vi "FuncVI_Sub - Script - Pass Parameters.vi"(6 "action":enum32{"import", "export"}(ring), 7 "Local VC Handle":T2, 8 "error in":errorcluster, 10 "parateters specifier":string, 11 "CE InstanceRef":T1) -> (0 "error out":errorcluster, 2 "dup parateters specifier":string, 3 "dup CE InstanceRef":T1, 5 "Local VC Handle out":T2)   [LabVIEW 2021]
doc: "::: CalcExpress Toolkit :::\nCopyright (c) 2000-2026 Konstantin Shifershteyn. All rights reserved."
uses:
  cetypes.llb/VarMan Variable Context Handle.ctl
  cetypes.llb/CalcExpress Instance RefNum.ctl
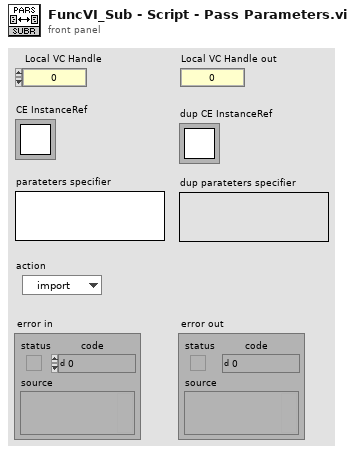
[diagram p1: front panel]
types:
  T1 = typedef "CalcExpress Instance RefNum.ctl" = refnum<k1>
  T2 = typedef "VarMan Variable Context Handle.ctl" = i32
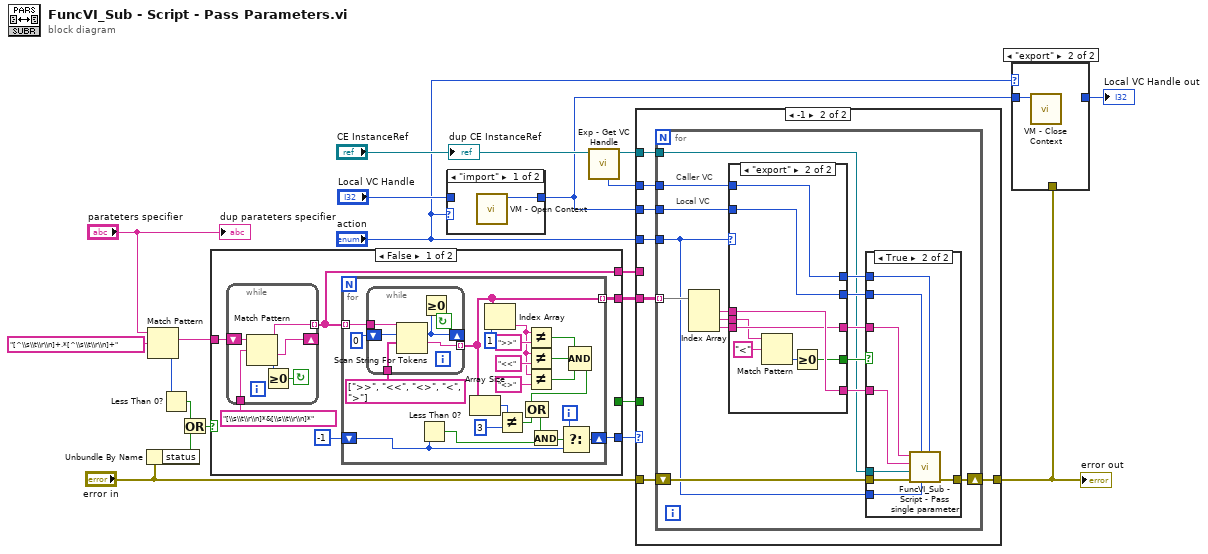
[diagram p0: block diagram]
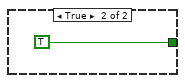
[diagram p4: hidden frame]
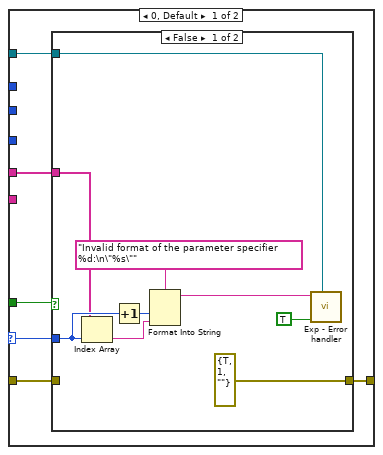
[diagram p5: hidden frame]
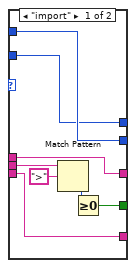
[diagram p8: hidden frame]
diagram:
  n1 = Unbundle By Name("error in") -> ("status"=w5:bool)
  n2 = Match Pattern(string="parateters specifier", regular expression="[^\\s\\t\\r\\n]+.*[^\\s\\t\\r\\n]+") -> (match substring=w1:string, offset past match=w7:i32)  [unwired: 1 in, 2 out]
  n3 = Less Than 0?(x=w7) -> (x < 0?=w6:bool)
  n4 = Or(x=w6, y=w5) -> (x .or. y?=w4:bool)
  n5 = case shown="False" w4 {
    tunnel: w1 -> [w25 _]
    tunnel: [w24 _] -> w20
    tunnel: [w23 _] -> w15
    tunnel: [_ TRUE] -> w19
    tunnel: [w21 _] -> w18
    frame False {
      n6 = while {
        tunnel: "[\\s\\t\\r\\n]*&[\\s\\t\\r\\n]*" -> [w60]
        shift-right: [w57] -> _
        shift-left: w25 -> [w59]
        tunnel: [w58] -> w21 mode=indexing
        stop <- w55 continue-if-true
        n7 = Match Pattern(string=w59, regular expression=w60) -> (before substring=w58:string, after substring=w57:string, offset past match=w56:i32)  [unwired: 1 in, 1 out]
        n8 = Greater Or Equal To 0?(x=w56) -> (x >= 0?=w55:bool)
      }
      n9 = for {
        tunnel: w21 -> [w41] mode=indexing
        shift-right: [w32] -> w24
        shift-left: -1 -> [w30]
        tunnel: [w35] -> w23 mode=indexing
        i -> [w31]
        n10 = while {
          tunnel: w41 -> [w54]
          shift-right: [w52] -> _
          shift-left: 0 ("offset past token") -> [w53]
          tunnel: [w50] -> w35 mode=indexing
          tunnel: string[] [">>", "<<", "<>", "<", ">"] ("operators (none)") -> [w49]
          stop <- w51 continue-if-true
          n11 = Scan String For Tokens(7:w49, 8:w53, 9:w54) -> (1:w50:string, 2:w52:i32)  [unwired: 3 in, 2 out]
          n12 = Greater Or Equal To 0?(x=w52) -> (x >= 0?=w51:bool)
        }
        n13 = Less Than 0?(x=w30) -> (x < 0?=w28:bool)
        n14 = Array Size(array=w35) -> (size(s)=w39:i32)
        n15 = Index Array(array=w35, index=1) -> (element=w34:string)
        n16 = Not Equal?(x=w39, y=3) -> (x != y?=w37:bool)
        n17 = Not Equal?(x=w34, y=">>") -> (x != y?=w46:bool)
        n18 = Not Equal?(x=w34, y="<<") -> (x != y?=w45:bool)
        n19 = Not Equal?(x=w34, y="<>") -> (x != y?=w42:bool)
        n20 = Compound Arithmetic op=AND(w46, w45, w42) -> (w44:bool)
        n21 = Compound Arithmetic op=OR(w44, w37) -> (w29:bool)
        n22 = And(x=w29, y=w28) -> (x .and. y?=w27:bool)
        n23 = Select(t=w31, s=w27, f=w30) -> (s? t:f=w32:i32)
      }
    }
    frame True {
    }
  }
  n24 = case shown="\"import\"" "action" {
    tunnel: [w62 w63] -> w11
    tunnel: "Local VC Handle" -> [_ w63]
    frame "import" {
      n25 = call "VM - Open Context.vi"() -> ("VC Handle out"=w62:T2)  [unwired: 9 in, 2 out]
    }
    frame "export" {
    }
  }
  n26 = call "Exp - Get VC Handle.vi"("InstanceRef"="CE InstanceRef") -> ("dup InstanceRef"=w14:T1, "VC Handle"=w12:T2)  [unwired: 5 in, 2 out]
  n27 = case shown="-1" w20 {
    selector: w20 -> [w66 _]
    tunnel: w15 -> [_ w86]
    tunnel: "error in" -> [w68 w85]
    tunnel: w12 -> [_ w84]
    tunnel: [w67 w83] -> w17
    tunnel: w19 -> [w69 _]
    tunnel: w18 -> [w65 _]
    tunnel: w14 -> [w64 w82]
    tunnel: "action" -> [_ w81]
    tunnel: w11 -> [_ w80]
    frame 0, Default {
      n28 = case shown="False" w69 {
        tunnel: w68 -> [_ w79]
        tunnel: [errorcluster {"status"=TRUE, "code"=1, "source"=""} ("error IO") w79] -> w67
        tunnel: w64 -> [w77 _]
        tunnel: w66 -> [w73 _]
        tunnel: w65 -> [w71 _]
        frame False {
          n29 = Index Array(array=w71, index=w73) -> (element=w72:string)
          n30 = Increment(x=w73) -> (x+1=w74:i32)
          n31 = Format Into String(format string="Invalid format of the parameter specifier %d:\n\"%s\"" ("error message in"), w74, w72) -> (resulting string=w70:string)  [unwired: 2 in, 1 out]
          n32 = call "Exp - Error handler.vi"("InstanceRef"=w77, "error in"=TRUE, "error message in"=w70) -> ()  [unwired: 6 in, 3 out]
        }
        frame True {
          # "INPUT ERROR\nor\nempty paramerers string"
        }
      }
    }
    frame -1 {
      n33 = for {
        shift-right: [w96] -> w83
        shift-left: w85 -> [w91]
        tunnel: w86 -> [w101] mode=indexing
        tunnel: w84 -> [w94]
        tunnel: w82 -> [w89]
        tunnel: w81 -> [w88]
        tunnel: w80 -> [w87]
        # "Local VC"
        # "Caller VC"
        n34 = Index Array(array=w101) -> (element #1=w100:string, element #2=w95:string, element #3=w98:string)  [unwired: 3 in]
        n35 = case shown="\"export\"" w88 {
          tunnel: w100 -> [w117 w126]
          tunnel: [w117 w125] -> w99
          tunnel: w98 -> [w118 w125]
          tunnel: [w118 w126] -> w97
          tunnel: w95 -> [w116 w121]
          tunnel: [w113 w122] -> w90
          tunnel: w94 -> [w112 w120]
          tunnel: w87 -> [w111 w119]
          tunnel: [w112 w119] -> w93
          tunnel: [w111 w120] -> w92
          frame "import" {
            n36 = Match Pattern(string=w116, regular expression=">") -> (offset past match=w114:i32)  [unwired: 1 in, 3 out]
            n37 = Greater Or Equal To 0?(x=w114) -> (x >= 0?=w113:bool)
          }
          frame "export" {
            n38 = Match Pattern(string=w121, regular expression="<") -> (offset past match=w123:i32)  [unwired: 1 in, 3 out]
            n39 = Greater Or Equal To 0?(x=w123) -> (x >= 0?=w122:bool)
          }
        }
        n40 = case shown="True" w90 {
          tunnel: w99 -> [_ w108]
          tunnel: w97 -> [_ w107]
          tunnel: [w102 w109] -> w96
          tunnel: w91 -> [w102 w110]
          tunnel: w93 -> [_ w106]
          tunnel: w92 -> [_ w105]
          tunnel: w89 -> [_ w104]
          tunnel: w88 -> [_ w103]
          frame False {
          }
          frame True {
            n41 = call "FuncVI_Sub - Script - Pass single parameter.vi"("Dst VC Handle"=w105, "action"=w103, "Src VC Handle"=w106, "error in"=w110, "CE InstanceRef"=w104, "Dst var name"=w107, "Src var name"=w108) -> ("error out"=w109:errorcluster)  [unwired: 4 in]
          }
        }
      }
    }
  }
  "error out" <- w17
  n42 = case shown="\"export\"" "action" {
    tunnel: w17 -> [_ _]
    tunnel: w11 -> [w127 w128]
    tunnel: [w127 _] -> w16
    frame "import" {
    }
    frame "export" {
      n43 = call "VM - Close Context.vi"("VC Handle"=w128) -> ()  [unwired: 9 in, 2 out]
    }
  }
  "Local VC Handle out" <- w16
  "dup CE InstanceRef" <- "CE InstanceRef"
  "dup parateters specifier" <- "parateters specifier"
